vi "Input Parameter Cluster Documentation--constant.vi"() -> (3 "Input Parameter Cluster Documentation":string)   [LabVIEW 2026]
doc: "This constant defines the documentation string of input parameter clusters (as a format string)."
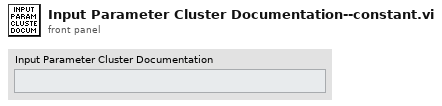
[diagram p1: front panel]
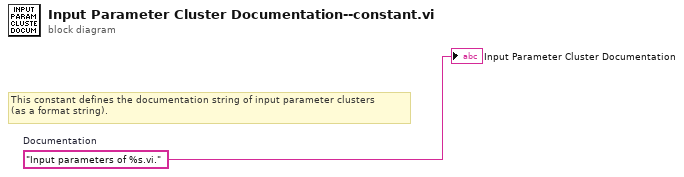
[diagram p0: block diagram]
diagram:
  w1 = "Input parameters of %s.vi."  # Documentation
  # "This constant defines the documentation string of input parameter clusters \n(as a format string)."
  "Input Parameter Cluster Documentation" <- w1
